vi "SerialOpen.vi"(1 "副本(F)":bool, 4 "Timeout":u32=1000, 5 "termination char":u8 caption="终止符" format="%.0x", 6 "Event Type":u32(ring) items=["禁用"=0, "服务请求"=1073684491, "触发"=3221168138, "清除"=1073684493, "VXI信号"=1073684512, "VXI/VME中断"=3221168161, "VXI/VME系统故障"=1073684509, "VXI/VME系统重启"=1073684510, "GPIB CIC"=1073684498, "GPIB通话"=1073684499, "GPIB侦听"=1073684500, "PXI干扰"=1073684514, "串口中断"=1073684515, "串口终止字符"=1073684516, "串口CTS"=1073684521, "串口DSR"=1073684522, "串口DCD"=1073684524, "串口RI"=1073684526, "串口字符"=1073684533, "USB中断"=1073684535, "全部启用"=1073709055], 7 "parity":enum16{"None", "Odd", "Even", "Mark", "Space"}(ring), 8 "error in (no error)":errorcluster caption="错误输入（无错误）", 9 "Data Bits":u16=8, 10 "Baud Rate":u32=9600, 11 "Port":refnum<visa-resource-name>) -> (0 "error out":errorcluster caption="错误输出", 3 "Port out":refnum<visa-resource-name>)   [LabVIEW 2025]
panel:
  in  "Stop Bits":u16(ring)=10 items=["1.0"=10, "1.5"=15, "2.0"=20]
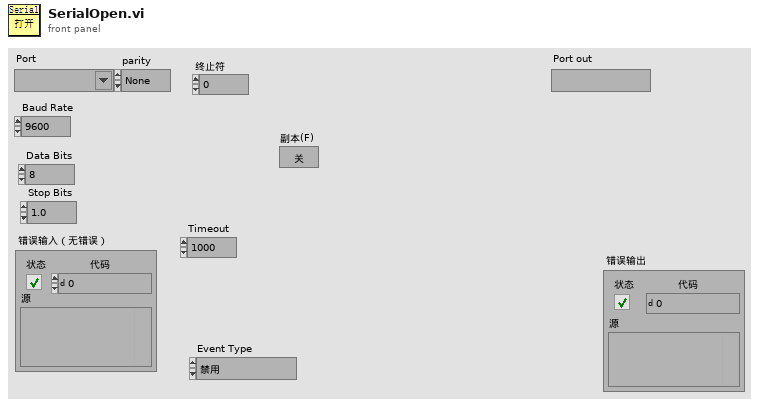
[diagram p1: front panel]
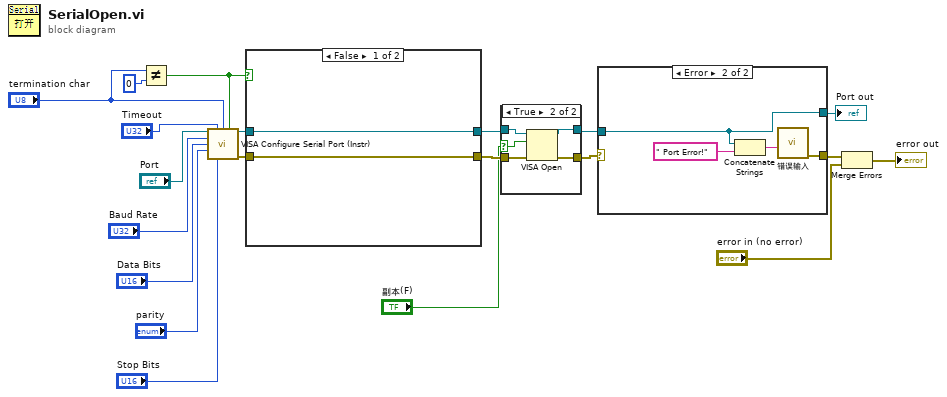
[diagram p0: block diagram]
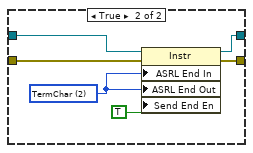
[diagram p3: hidden frame]
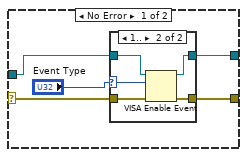
[diagram p4: hidden frame]
diagram:
  n1 = Not Equal?(x="termination char", y=u8 0) -> (x != y?=w2:bool)
  n2 = call <vilib>:"VISA Configure Serial Port (Instr).vi"("VISA resource name"="Port", "timeout (10sec)"="Timeout", "termination char\n(0xA = '\\n' = LF)"="termination char", "Enable Termination\nChar (T)"=w2, "baud rate (9600)"="Baud Rate", "data bits (8)"="Data Bits", "parity (0:none)"="parity", "stop bits (10: 1 bit)"="Stop Bits") -> ("VISA resource name out"=w14:refnum<visa-resource-name>, "error out"=w11:errorcluster)  [unwired: 6 in]
  n3 = case shown="False" w2 {
    tunnel: w14 -> [w22 w28]
    tunnel: [w22 w27] -> w13
    tunnel: [w21 w26] -> w12
    tunnel: w11 -> [w21 w25]
    frame False {
    }
    frame True {
      w24 = u16 2 items=["None", "LastBit", "TermChar"] ("Serial Settings:Serial End Mode for Reads")
      n4 = property class="Instr"(reference=w28, error in=w25, "ASRL End In"=w24, "ASRL End Out"=w24, "Send End En"=TRUE ("Serial Settings:Allow Transmit")) -> (reference out=w27:refnum<visa-resource-name>, error out=w26:errorcluster)
    }
  }
  n5 = case shown="True" "副本(F)" {
    selector: "副本(F)" -> [_ w31]
    tunnel: [w30 w35] -> w16
    tunnel: [w29 w34] -> w15
    tunnel: w13 -> [w30 w33]
    tunnel: w12 -> [w29 w32]
    frame False {
    }
    frame True {
      n6 = VISA Open(duplicate session (F)=w31, error in (no error)=w32, VISA resource name=w33) -> (VISA resource name=w35:refnum<visa-resource-name>, error out=w34:errorcluster)  [unwired: 2 in]
    }
  }
  n7 = case shown="Error" w15 {
    selector: w15 -> [w40 _]
    tunnel: [w39 w49] -> w17
    tunnel: w16 -> [w38 w48]
    tunnel: [w36 w48] -> w18
    frame No Error {
      n8 = case shown="1.." "Event Type" {
        selector: "Event Type" -> [_ w45]
        tunnel: w40 -> [w42 w47]
        tunnel: [w42 w46] -> w39
        tunnel: w38 -> [w41 w44]
        tunnel: [w41 w43] -> w36
        frame 0, Default {
        }
        frame 1.. {
          n9 = VISA Enable Event(8:w47, 10:w45, 11:w44) -> (0:w46:errorcluster, 3:w43:refnum<visa-resource-name>)  [unwired: 1 in]
        }
      }
    }
    frame Error {
      n10 = Concatenate Strings(w48, " Port Error!" ("字符串")) -> (w50:string)
      n11 = call "错误输入.vi"("source"=w50) -> ("error out"=w49:errorcluster)  [unwired: 10 in]
    }
  }
  "Port out" <- w18
  n12 = Merge Errors(w17, "error in (no error)") -> (→"error out":errorcluster)
